vi "Search_index.vi"(8 "error in (no error)":errorcluster caption="错误输入（无错误）", 10 "ID":string, 11 "Procotol_class 输入":refnum<class "Procotol_class.lvclass">) -> (0 "error out":errorcluster caption="错误输出", 1 "numb_index":i32, 2 "ARR_index":i32[](array[numeric]), 3 "Procotol_class 输出":refnum<class "Procotol_class.lvclass">)   [LabVIEW 2025, in "Procotol_class.lvclass"]
uses:
  Procotol_class.lvclass
  Procotol_class.lvclass/Procotol_class.ctl
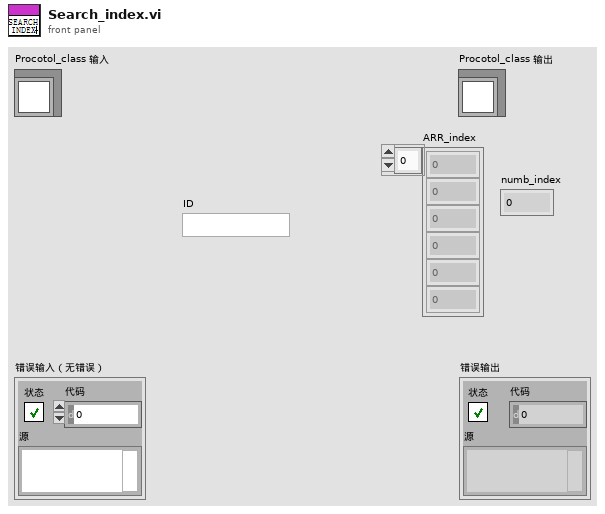
[diagram p1: front panel]
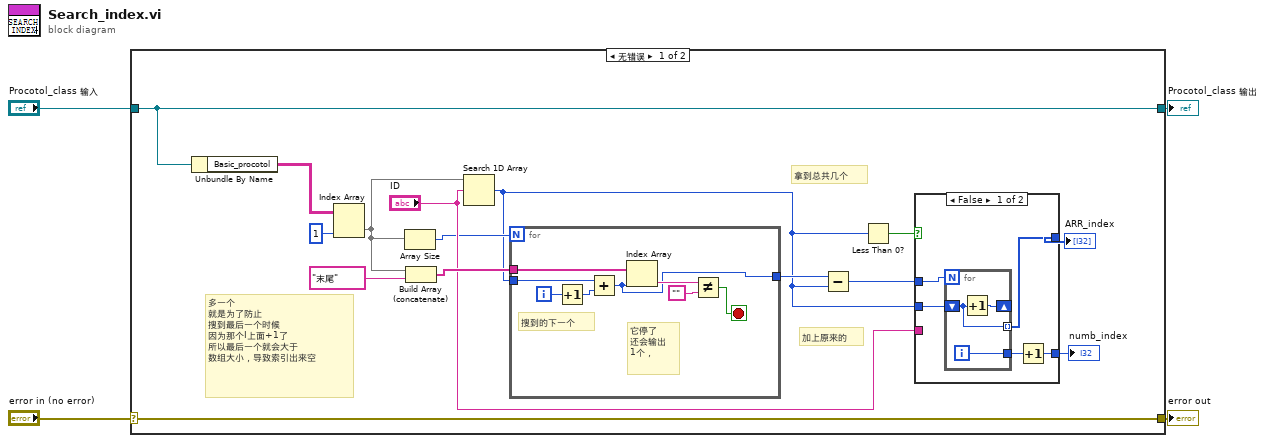
[diagram p0: block diagram]
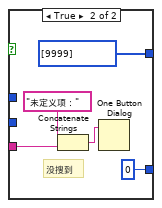
[diagram p2: hidden frame]
diagram:
  n1 = case shown="无错误" "error in (no error)" {
    selector: "error in (no error)" -> [w19 w42]
    tunnel: [w19 w42] -> w3
    tunnel: [w18 w41] -> w1
    tunnel: "Procotol_class 输入" -> [w18 w41]
    frame No Error {
      # "加上原来的"
      # "拿到总共几个"
      # "多一个\n就是为了防止\n搜到最后一个时候\n因为那个I上面+1了\n所以最后一个就会大于\n数组大小，导致索引出来空"
      n2 = Unbundle By Name(w18) -> ("Basic_procotol"=w6:string[][])
      n3 = Index Array(array=w6, index (col)=1 ("禁用的索引 (列)")) -> (element=w13:string[])  [unwired: 1 in]
      n4 = Array Size(array=w13) -> (size(s)=w9:i32)
      n5 = Build Array (concatenate)(w13, "末尾" ("元素")) -> (w14:string[])
      n6 = Search 1D Array(1D array=w13, element="ID") -> (index of element=w7:i32)  [unwired: 1 in]
      n7 = for {
        N: w9 -> [_]
        tunnel: w14 -> [w27]
        tunnel: w7 -> [w26]
        tunnel: [w22] -> w11
        i -> [w25]
        stop <- w20 stop-if-true
        # "它停了\n还会输出\n1个，"
        # "搜到的下一个"
        n8 = Increment(x=w25) -> (x+1=w23:i32)
        n9 = Add(x=w26, y=w23) -> (x+y=w22:i32)
        n10 = Index Array(array=w27, index=w22) -> (element=w24:string)
        n11 = Not Equal?(x=w24, y="") -> (x != y?=w20:bool)
      }
      n12 = Subtract(x=w11, y=w7) -> (x-y=w10:i32)
      n13 = Less Than 0?(x=w7) -> (x < 0?=w8:bool)
      n14 = case shown="False" w8 {
        tunnel: [w30 i32[] [9999]] -> w16
        tunnel: "ID" -> [_ w37]
        tunnel: w10 -> [w32 _]
        tunnel: w7 -> [w31 _]
        tunnel: [w28 0] -> w5
        frame False {
          n15 = for {
            N: w32 -> [_]
            shift-right: [w35] -> _
            shift-left: w31 -> [w34]
            tunnel: [w34] -> w30 mode=indexing
            tunnel: [w33] -> w29
            i -> [w33]
            n16 = Increment(x=w34) -> (x+1=w35:i32)
          }
          n17 = Increment(x=w29) -> (x+1=w28:i32)
        }
        frame True {
          # "没搜到"
          n18 = Concatenate Strings("未定义项：", w37) -> (w38:string)
          n19 = One Button Dialog(message=w38) -> ()  [unwired: 1 in, 1 out]
        }
      }
      "ARR_index" <- w16
      "numb_index" <- w5
    }
    frame Error {
    }
  }
  "error out" <- w3
  "Procotol_class 输出" <- w1
